vi "measure Average Power Measurement.vi"(8 "error in (no error)":errorcluster, 11 "SA Measurement in":refnum<class "SA Measurement.lvclass">) -> (0 "error out":errorcluster, 2 "Channel Power":dbl, 3 "SA Measurement out":refnum<class "SA Measurement.lvclass">)   [LabVIEW 2023, in "Spectrum Analyzer.lvlib" / "SA Measurement.lvclass"]
uses:
  SA Measurement.lvclass
  SA Measurement.lvclass/SA Measurement.ctl
  TYPE DEFINITION/Keysight 9020A/TYPE Measurement Preset.ctl
  Spectrum Analyzer.lvlib
  TYPE DEFINITION/TYPE RBW and VBW Select.ctl
  Interface_Spectrum/Interface_Spectrum.lvclass
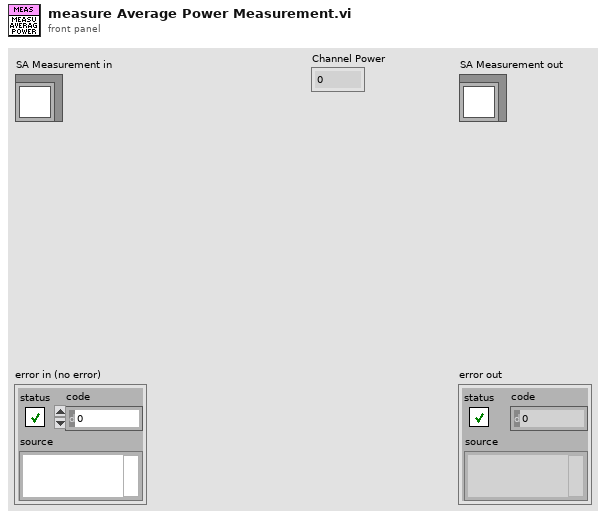
[diagram p1: front panel]
types:
  T1 = typedef "Spectrum Analyzer.lvlib/TYPE RBW and VBW Select.ctl" = enum16{"Res BW", "Video BW"}
  T2 = typedef "Spectrum Analyzer.lvlib/TYPE Measurement Preset.ctl" = enum16{"Sweep SA Mode", "Channel Power", "Occupied BW", "ACP", "Spurious Emission", "Spurious Emission Mask", "Burst Power (Transmit Power)"}
  T3 = typedef "Spectrum Analyzer.lvlib/TYPE Y-axis Unit.ctl" = enum16{"dBm", "dBmV", "dBuV", "dBpW", "Volt", "Ampere", "Watt"}
  T4 = typedef "Spectrum Analyzer.lvlib/TYPE Reference Level and Atten Param.ctl" = cluster{"Reference Level":dbl, "Atten":i32, "Atten Auto?":bool, "Reference Level Offset":dbl}
  T5 = typedef "Spectrum Analyzer.lvlib/TYPE Display Trace Mode Select.ctl" = enum16{"Clear Write", "Max Hold", "Min Hold", "Average", "View"}
  T6 = typedef "Spectrum Analyzer.lvlib/TYPE Detect Mode Select.ctl" = enum16{"Det Auto (Normal)", "Auto Peak", "Positive Peak", "Negative Peak", "Sample", "RMS", "Average", "Quasipeak", "CISPR Average", "RMS Average"}
  T7 = cluster{"Trace Mode":T5, "Detector Type":T6, "Detect Auto?":bool}[]
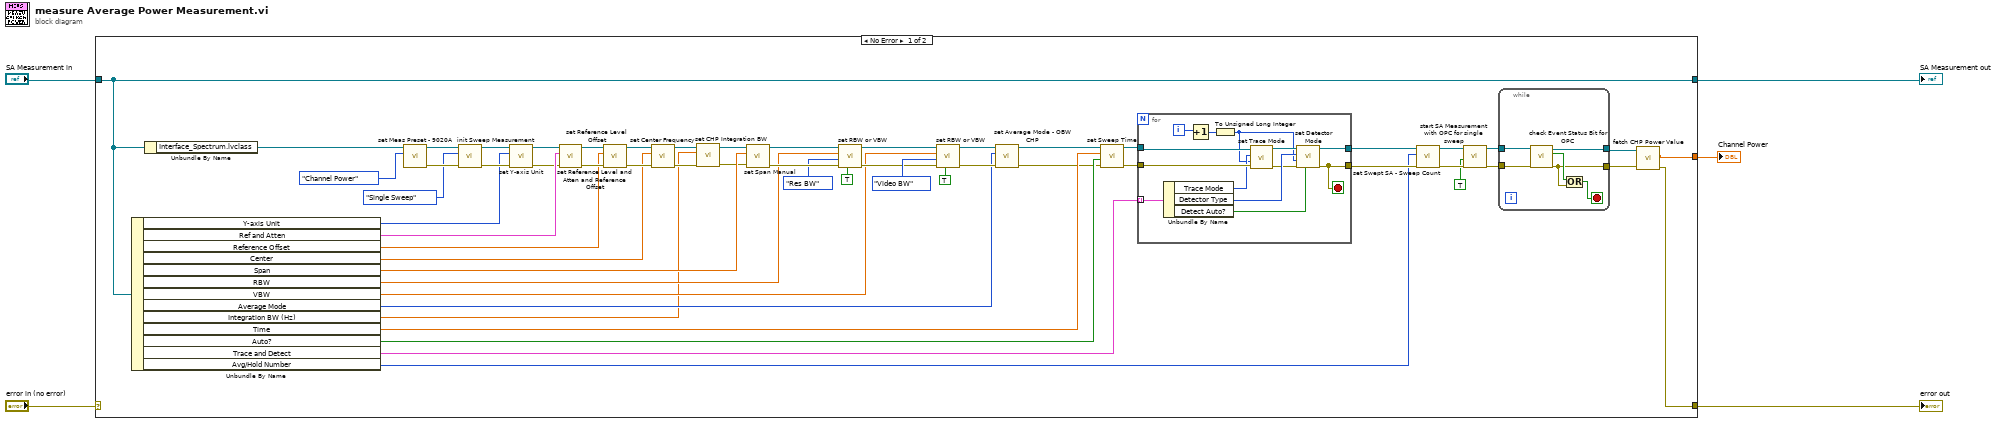
[diagram p0: block diagram]
diagram:
  n1 = case shown="No Error" "error in (no error)" {
    selector: "error in (no error)" -> [_ w82]
    tunnel: [w14 w82] -> w4
    tunnel: [w20 w81] -> w2
    tunnel: "SA Measurement in" -> [w20 w81]
    tunnel: [w13 _] -> w1
    frame No Error {
      n2 = Unbundle By Name(w20) -> ("Y-axis Unit"=w34:T3, "Ref and Atten"=w56:T4, "Reference Offset"=w53:dbl, "Center"=w50:dbl, "Span"=w49:dbl, "RBW"=w46:dbl, "VBW"=w39:dbl, "Average Mode"=w17:enum16{"Exponential", "Repeat"}, "Integration BW (Hz)"=w8:dbl, "Time"=w33:dbl, "Auto?"=w32:bool, "Trace and Detect"=w29:T7, "Avg/Hold Number"=w26:u32)
      n3 = Unbundle By Name(w20) -> ("Interface_Spectrum.lvclass"=w61:refnum<class "Interface_Spectrum.lvclass">)
      n4 = call-dynamic "set Meas Preset - 9020A.vi"("Measurement Preset"=TYPE_Measurement_Preset."Channel Power", "Interface_Spectrum in"=w61) -> ("error out"=w58:errorcluster, "Interface_Spectrum out"=w59:refnum<class "Interface_Spectrum.lvclass">)  [unwired: 8 in]
      n5 = call-dynamic "init Sweep Measurement.vi"("error in (no error)"=w58, "Sweep Measurement Mode"=enum16{"Single Sweep", "Continuous Sweep"}."Single Sweep", "Interface_Spectrum in"=w59) -> ("error out"=w37:errorcluster, "Interface_Spectrum out"=w38:refnum<class "Interface_Spectrum.lvclass">)  [unwired: 7 in]
      n6 = call-dynamic "set Y-axis Unit.vi"("error in (no error)"=w37, "Y-axis Unit"=w34, "Interface_Spectrum in"=w38) -> ("error out"=w35:errorcluster, "Interface_Spectrum out"=w36:refnum<class "Interface_Spectrum.lvclass">)  [unwired: 7 in]
      n7 = call-dynamic "set Reference Level and Atten and Reference Offset.vi"("error in (no error)"=w35, "Reference Level, Atten, Reference Offset"=w56, "Interface_Spectrum in"=w36) -> ("error out"=w54:errorcluster, "Interface_Spectrum out"=w55:refnum<class "Interface_Spectrum.lvclass">)  [unwired: 7 in]
      n8 = call-dynamic "set Reference Level Offset.vi"("error in (no error)"=w54, "Reference Level Offset"=w53, "Interface_Spectrum in"=w55) -> ("error out"=w51:errorcluster, "Interface_Spectrum out"=w52:refnum<class "Interface_Spectrum.lvclass">)  [unwired: 7 in]
      n9 = call-dynamic "set Center Frequency.vi"("error in (no error)"=w51, "Center Frequency (Hz)"=w50, "Interface_Spectrum in"=w52) -> ("error out"=w11:errorcluster, "Interface_Spectrum out"=w12:refnum<class "Interface_Spectrum.lvclass">)  [unwired: 7 in]
      n10 = call-dynamic "set CHP Integration BW.vi"("error in (no error)"=w11, "Integration BW (Hz)"=w8, "Interface_Spectrum in"=w12) -> ("error out"=w9:errorcluster, "Interface_Spectrum out"=w10:refnum<class "Interface_Spectrum.lvclass">)  [unwired: 7 in]
      n11 = call-dynamic "set Span Manual.vi"("error in (no error)"=w9, "Span (Hz)"=w49, "Interface_Spectrum in"=w10) -> ("error out"=w47:errorcluster, "Interface_Spectrum out"=w48:refnum<class "Interface_Spectrum.lvclass">)  [unwired: 7 in]
      n12 = call-dynamic "set RBW or VBW.vi"("BW Auto?"=TRUE, "error in (no error)"=w47, "BW Type"=TYPE_RBW_and_VBW_Select."Res BW", "BW Value (Hz)"=w46, "Interface_Spectrum in"=w48) -> ("error out"=w40:errorcluster, "Interface_Spectrum out"=w41:refnum<class "Interface_Spectrum.lvclass">)  [unwired: 5 in]
      n13 = call-dynamic "set RBW or VBW.vi"("BW Auto?"=TRUE, "error in (no error)"=w40, "BW Type"=TYPE_RBW_and_VBW_Select."Video BW", "BW Value (Hz)"=w39, "Interface_Spectrum in"=w41) -> ("error out"=w18:errorcluster, "Interface_Spectrum out"=w19:refnum<class "Interface_Spectrum.lvclass">)  [unwired: 5 in]
      n14 = call-dynamic "set Average Mode - OBW CHP.vi"("error in (no error)"=w18, "Average Mode"=w17, "Interface_Spectrum in"=w19) -> ("error out"=w6:errorcluster, "Interface_Spectrum out"=w7:refnum<class "Interface_Spectrum.lvclass">)  [unwired: 7 in]
      n15 = call-dynamic "set Sweep Time.vi"("error in (no error)"=w6, "Sweep Time Auto?"=w32, "Sweep Time(sec)"=w33, "Interface_Spectrum in"=w7) -> ("error out"=w30:errorcluster, "Interface_Spectrum out"=w31:refnum<class "Interface_Spectrum.lvclass">)  [unwired: 6 in]
      n16 = for {
        tunnel: w31 -> [w79]
        tunnel: w30 -> [w78]
        tunnel: w29 -> [w80] mode=indexing
        tunnel: [w68] -> w27
        tunnel: [w69] -> w28
        i -> [w77]
        stop <- w68 stop-if-true
        n17 = Unbundle By Name(w80) -> ("Trace Mode"=w75:T5, "Detector Type"=w73:T6, "Detect Auto?"=w70:bool)
        n18 = Increment(x=w77) -> (x+1=w76:i32)
        n19 = To Unsigned Long Integer(number=w76) -> (unsigned 32bit integer=w71:u32)
        n20 = call-dynamic "set Trace Mode.vi"("error in (no error)"=w78, "Trace Index"=w71, "Trace Mode"=w75, "Interface_Spectrum in"=w79) -> ("error out"=w72:errorcluster, "Interface_Spectrum out"=w74:refnum<class "Interface_Spectrum.lvclass">)  [unwired: 6 in]
        n21 = call-dynamic "set Detector Mode.vi"("Detect Auto?"=w70, "error in (no error)"=w72, "Trace Index"=w71, "Detector Type"=w73, "Interface_Spectrum in"=w74) -> ("error out"=w68:errorcluster, "Interface_Spectrum out"=w69:refnum<class "Interface_Spectrum.lvclass">)  [unwired: 5 in]
      }
      n22 = call-dynamic "set Swept SA - Sweep Count.vi"("error in (no error)"=w27, "Sweep Count"=w26, "Interface_Spectrum in"=w28) -> ("error out"=w24:errorcluster, "Interface_Spectrum out"=w25:refnum<class "Interface_Spectrum.lvclass">)  [unwired: 7 in]
      n23 = call-dynamic "start SA Measurement with OPC for single sweep.vi"("error in (no error)"=w24, "with OPC?"=TRUE, "Interface_Spectrum in"=w25) -> ("error out"=w21:errorcluster, "Interface_Spectrum out"=w22:refnum<class "Interface_Spectrum.lvclass">)  [unwired: 7 in]
      n24 = while {
        tunnel: w22 -> [w67]
        tunnel: w21 -> [w66]
        tunnel: [w63] -> w15
        tunnel: [w62] -> w16
        stop <- w64 stop-if-true
        n25 = call-dynamic "check Event Status Bit for OPC.vi"("error in (no error)"=w66, "Interface_Spectrum in"=w67) -> ("error out"=w63:errorcluster, "OPC Bit Changed?"=w65:bool, "Interface_Spectrum out"=w62:refnum<class "Interface_Spectrum.lvclass">)  [unwired: 7 in]
        n26 = Or(x=w65, y=w63) -> (x .or. y?=w64:bool)
      }
      n27 = call-dynamic "fetch CHP Power Value.vi"("error in (no error)"=w15, "Interface_Spectrum in"=w16) -> ("error out"=w14:errorcluster, "Channel Power"=w13:dbl)  [unwired: 7 in, 1 out]
    }
    frame Error {
    }
  }
  "error out" <- w4
  "SA Measurement out" <- w2
  "Channel Power" <- w1
